vi "Set Column Value.vi"(7 "Column":i32, 9 "Value":string, 10 "Row In":string[](array[string]), 11 "Result Handler":refnum<class "TestStand Result Handler.lvclass">) -> (2 "Row Out":string[](array[string]), 3 "Result Handler Out":refnum<class "TestStand Result Handler.lvclass">)   [LabVIEW 2020, in "Astemes_CSVReportPlugin.lvlib" / "TestStand Result Handler.lvclass"]
uses:
  TestStand Result Handler.lvclass
  TestStand Result Handler.lvclass/TestStand Result Handler.ctl
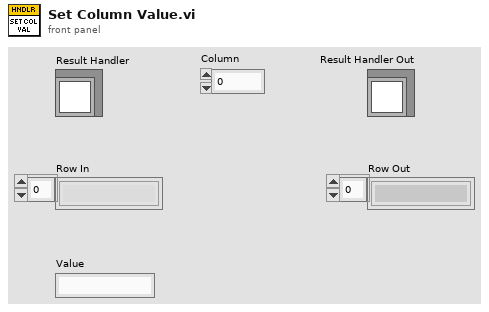
[diagram p1: front panel]
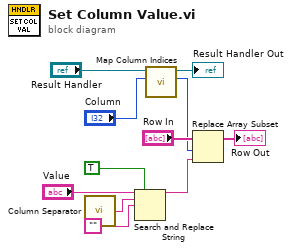
[diagram p0: block diagram]
diagram:
  n1 = call "Column Separator.vi"() -> ("delimiter"=w7:string)
  n2 = Search and Replace String(replace all?=TRUE ("replace all? (F)"), input string="Value", search string=w7, replace string="" ("replace string (\"\")")) -> (result string=w8:string)  [unwired: 4 in, 3 out]
  n3 = call-dynamic "Map Column Indices.vi"("Index"="Column", "TestStand Result Handler in"="Result Handler") -> ("Mapped Index"=w2:i32, "TestStand Result Handler out"=→"Result Handler Out":refnum<class "TestStand Result Handler.lvclass">)  [unwired: 7 in, 1 out]
  n4 = Replace Array Subset(array="Row In", new element=w8, index=w2) -> (→"Row Out":string[])
